vi "UI_Draw_Tiles.vi"(0 "Picture":picture, 5 "Channels":T1(array[cluster]), 7 "Running":bool, 9 "Phase":bool, 11 "error in":errorcluster) -> (4 "New Picture":picture, 15 "error out":errorcluster)   [LabVIEW 2026]
doc: "128채널 타일 바둑판. 채널 i -> 열 i/8 (C섀시·M모듈), 행 i%8 (ai0~7)."
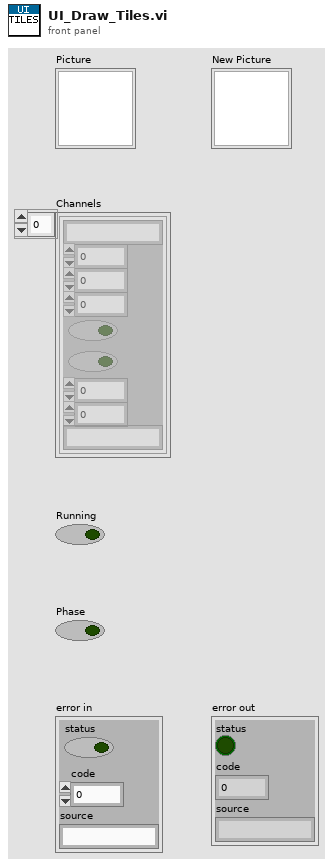
[diagram p1: front panel]
types:
  T1 = cluster{"Name":string, "Value":dbl, "High Limit":dbl, "Low Limit":dbl, "Save":bool, "Graph":bool, "Scale Min":dbl, "Scale Max":dbl, "Unit":string}[]
  T2 = cluster{"left":i16, "top":i16, "right":i16, "bottom":i16}
  T3 = cluster{"Font Name:":string, "Size":i16, "Strikeout?":bool, "Italic?":bool, "Underline?":bool, "Outline?":bool, "Shadow?":bool, "Bold?":bool}
  T4 = enum16{"User-specified Font", "Application Font", "System Font", "Dialog Font"}
  T5 = cluster{"horizontal":enum16{"left", "center", "right"}, "vertical":enum16{"top", "center", "bottom"}}
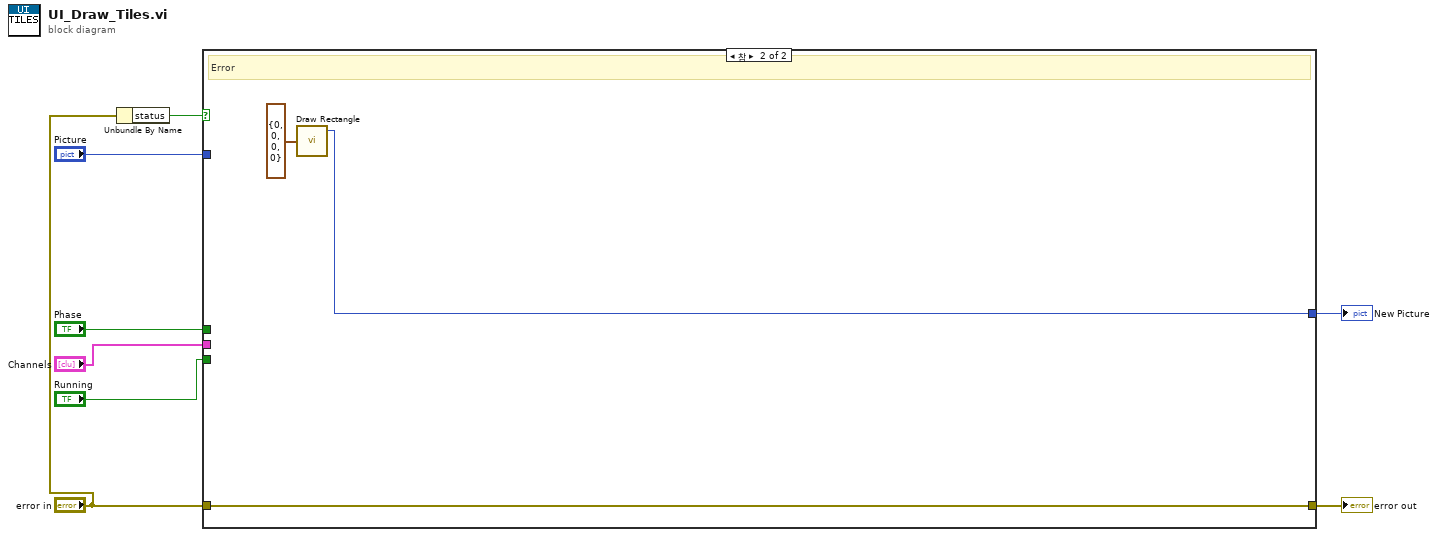
[diagram p0: block diagram]
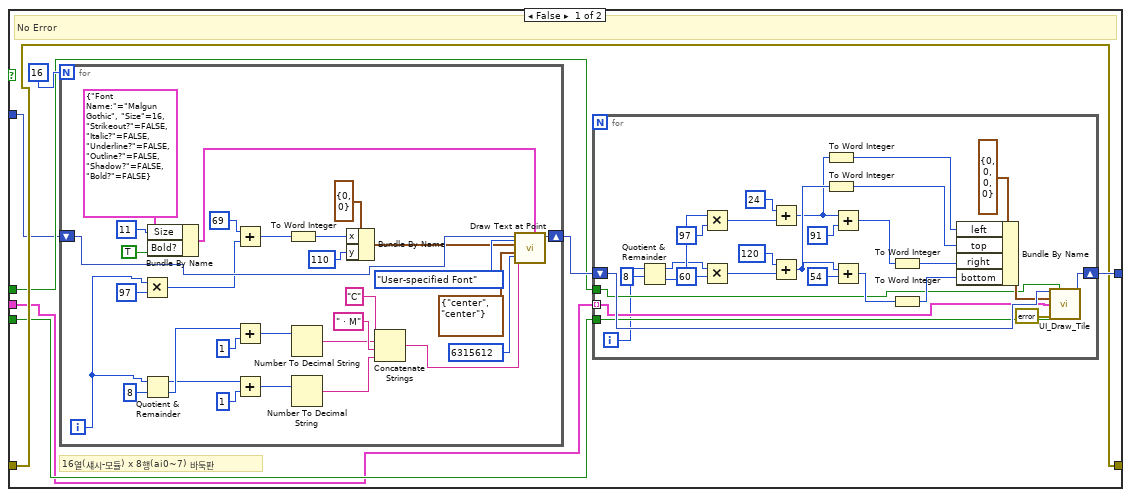
[diagram p2: hidden frame]
diagram:
  n1 = Unbundle By Name("error in") -> ("status"=w6:bool)
  n2 = case shown="참" w6 {
    tunnel: "Picture" -> [w9 _]
    tunnel: "Channels" -> [w10 _]
    tunnel: "Running" -> [w11 _]
    tunnel: "Phase" -> [w12 _]
    tunnel: "error in" -> [w13 w75]
    tunnel: [w13 w75] -> w8
    tunnel: [w16 w77] -> w7
    frame False {
      # "16열(섀시-모듈) x 8행(ai0~7) 바둑판"
      # "No Error"
      n3 = for {
        N: 16 -> [_]
        shift-right: [w73] -> w15
        shift-left: w9 -> [w74]
        i -> [w45]
        n4 = Multiply(x=w45, y=97) -> (x*y=w60:i32)
        n5 = Quotient & Remainder(x=w45, y=8) -> (x-y*floor(x/y)=w47:i32, floor(x/y)=w48:i32)
        n6 = Bundle By Name(cluster=T3 {"Font Name:"="Malgun Gothic", "Size"=16, "Strikeout?"=FALSE, "Italic?"=FALSE, "Underline?"=FALSE, "Outline?"=FALSE, "Shadow?"=FALSE, "Bold?"=FALSE}, "Size"=i16 11, "Bold?"=TRUE) -> (w72:T3)
        n7 = Add(x=69, y=w60) -> (x+y=w61:i32)
        n8 = Add(x=w48, y=1) -> (x+y=w51:i32)
        n9 = Add(x=w47, y=1) -> (x+y=w55:i32)
        n10 = To Word Integer(number=w61) -> (16bit integer=w62:i16)
        n11 = Number To Decimal String(number=w51) -> (decimal integer string=w52:string)  [unwired: 1 in]
        n12 = Number To Decimal String(number=w55) -> (decimal integer string=w56:string)  [unwired: 1 in]
        n13 = Bundle By Name(cluster=cluster{"x":i16, "y":i16} {"x"=0, "y"=0}, "x"=w62, "y"=i16 110) -> (w68:cluster{"x":i16, "y":i16})
        n14 = Concatenate Strings("C", w52, " · M", w56) -> (w57:string)
        n15 = call <vilib>:"Draw Text at Point.vi"("[user-specified font]"=w72, "text color(black)"=u32 6315612, "desired font(Application)"=T4."User-specified Font", "text"=w57, "alignment(left, top)"=T5 {"horizontal"=enum."center", "vertical"=enum."center"}, "origin"=w68, "picture"=w74) -> ("new picture"=w73:picture)  [unwired: 3 in, 1 out]
      }
      n16 = for {
        tunnel: w11 -> [w18]
        tunnel: w12 -> [w19]
        tunnel: w10 -> [w20] mode=indexing
        shift-right: [w43] -> w16
        shift-left: w15 -> [w44]
        i -> [w17]
        n17 = Quotient & Remainder(x=w17, y=8) -> (x-y*floor(x/y)=w22:i32, floor(x/y)=w23:i32)
        n18 = Multiply(x=w23, y=97) -> (x*y=w26:i32)
        n19 = Multiply(x=w22, y=60) -> (x*y=w30:i32)
        n20 = Add(x=24, y=w26) -> (x+y=w27:i32)
        n21 = Add(x=120, y=w30) -> (x+y=w31:i32)
        n22 = To Word Integer(number=w27) -> (16bit integer=w37:i16)
        n23 = To Word Integer(number=w31) -> (16bit integer=w38:i16)
        n24 = Add(x=w27, y=91) -> (x+y=w33:i32)
        n25 = Add(x=w31, y=54) -> (x+y=w35:i32)
        n26 = To Word Integer(number=w33) -> (16bit integer=w39:i16)
        n27 = To Word Integer(number=w35) -> (16bit integer=w40:i16)
        n28 = Bundle By Name(cluster=T2 {"left"=0, "top"=0, "right"=0, "bottom"=0}, "left"=w37, "top"=w38, "right"=w39, "bottom"=w40) -> (w41:T2)
        n29 = call "UI_Draw_Tile.vi"("Picture"=w44, "Phase"=w19, "Rect"=w41, "Channel"=w20, "Running"=w18, "error in"=errorcluster {"status"=FALSE, "code"=0, "source"=""}) -> ("New Picture"=w43:picture)  [unwired: 8 in, 1 out]
      }
    }
    frame True {
      # "Error"
      n30 = call <vilib>:"Draw Rectangle.vi"("rect"=T2 {"left"=0, "top"=0, "right"=0, "bottom"=0}) -> ("new picture"=w77:picture)  [unwired: 8 in]
    }
  }
  "New Picture" <- w7
  "error out" <- w8
